vi "Create.vi"(6 "Labels":map{string, string}(c390), 7 "Registry Name":string="_default_registry", 8 "error in (no error)":errorcluster) -> (0 "error out":errorcluster, 3 "LabVIEW Collector out":refnum<class "LabVIEW Collector.lvclass">)   [LabVIEW 2020, in "Collector.lvlib" / "LabVIEW Collector.lvclass"]
doc: "Default LabVIEW collector. Creates metrics about the LabVIEW application hosting this code."
uses:
  LabVIEW Collector.lvclass
  metrics/gauge/Gauge.lvclass
  C:/Github-locals/PromVIEW/src/metrics/metric/Metric.lvclass
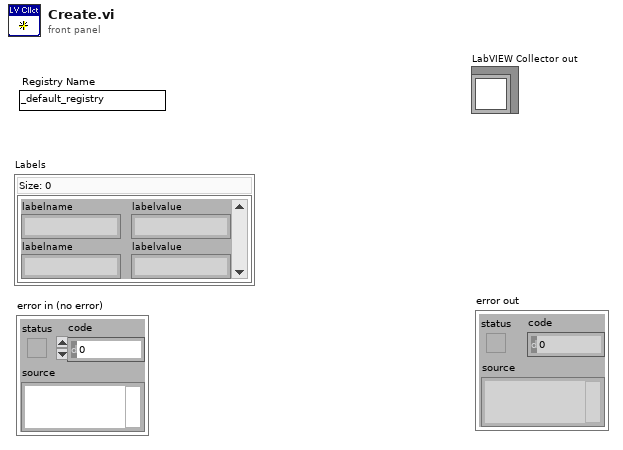
[diagram p1: front panel]
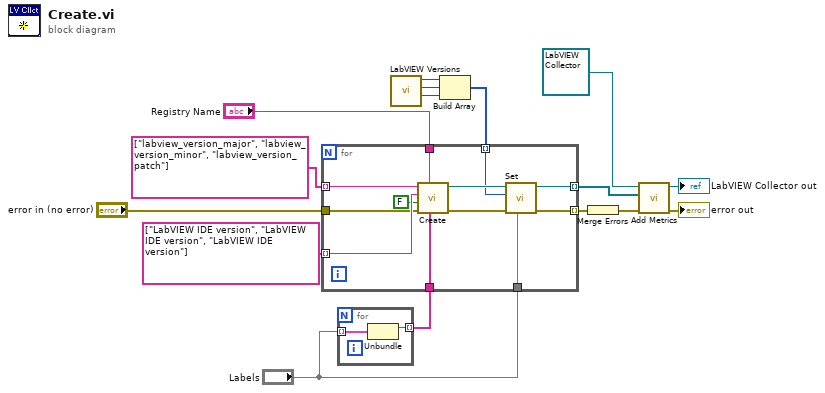
[diagram p0: block diagram]
diagram:
  n1 = for {
    tunnel: "Labels" -> [w18] mode=indexing
    tunnel: [w17] -> w2 mode=indexing
    n2 = Unbundle(w18) -> ("labelname"=w17:string)  [unwired: 1 out]
  }
  n3 = call "LabVIEW Versions.vi"() -> ("Patch"=w13:i32, "Minor"=w14:i32, "Major"=w15:i32)  [unwired: 9 in]
  n4 = Build Array(w15, w14, w13) -> (w12:i32[])
  n5 = for {
    tunnel: string[] ["labview_version_major", "labview_version_minor", "labview_version_patch"] ("Metric Name") -> [w29] mode=indexing
    tunnel: w12 -> [w28] mode=indexing
    tunnel: string[] ["LabVIEW IDE version", "LabVIEW IDE version", "LabVIEW IDE version"] ("Metric Name") -> [w27] mode=indexing
    tunnel: "Registry Name" -> [w26]
    tunnel: [w25] -> w9 mode=indexing
    tunnel: [w24] -> w7 mode=indexing
    tunnel: "error in (no error)" -> [w23]
    tunnel: w2 -> [w20]
    tunnel: "Labels" -> [w19]
    n6 = call "Create.vi"("Label Names"=w20, "Registry Name"=w26, "error in (no error)"=w23, "Auto-register?"=FALSE, "Description"=w27, "Metric Name"=w29) -> ("error out"=w22:errorcluster, "Gauge Ref"=w30:refnum<data-value>)  [unwired: 4 in]
    n7 = call "Set.vi"("Labels"=w19, "error in (no error)"=w22, "Value"=w28, "Gauge Ref"=w30) -> ("error out"=w24:errorcluster, "Gauge Ref out"=w25:refnum<data-value>)  [unwired: 6 in]
  }
  n8 = Merge Errors(w7) -> (w6:errorcluster)
  n9 = call-dynamic "Add Metrics.vi"("error in (no error)"=w6, "Metrics"=w9, "Default Collector in"=refnum<class "LabVIEW Collector.lvclass"> refnum ("Collector.lvlib:LabVIEW Collector.lvclass")) -> ("error out"=→"error out":errorcluster, "Default Collector out"=→"LabVIEW Collector out":refnum<class "LabVIEW Collector.lvclass">)  [unwired: 7 in]
